vi "Touch.vi"(8 "error in":errorcluster, 11 "Cls in":refnum<class "Cls.lvclass">) -> (0 "error out":errorcluster, 3 "Cls out":refnum<class "Cls.lvclass">)   [LabVIEW 2026, in "Cls.lvclass"]
doc: "Repro method: passes the object through."
uses:
  Cls.lvclass
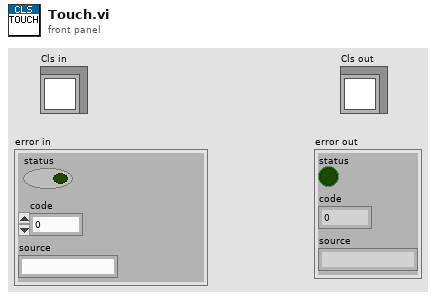
[diagram p1: front panel]
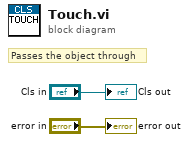
[diagram p0: block diagram]
diagram:
  # "Passes the object through"
  "Cls out" <- "Cls in"
  "error out" <- "error in"
